vi "Get Modification Flags.vi"(8 "error in (no error)":errorcluster, 10 "Saved Item in":refnum<class "Item.lvclass">, 11 "Item in":refnum<class "Item.lvclass">) -> (0 "error out":errorcluster, 1 "Modification Flags":bool[](array[boolean]), 2 "Saved Item out":refnum<class "Item.lvclass">, 3 "Item out":refnum<class "Item.lvclass">)   [LabVIEW 2020, in "VI Properties Editor.lvlib" / "Item.lvclass"]
doc: "Gets the modification flags of <B>Item in</B> by comparing it to <B>Saved Item in</B>."
uses:
  Item.lvclass
  <vilib>/LabVIEW Icon API/lv_icon/Classes/Icon/Icon.lvclass
  Item.lvclass/Item.ctl
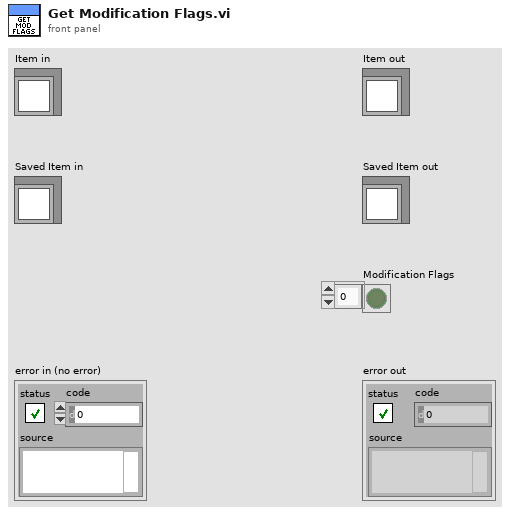
[diagram p1: front panel]
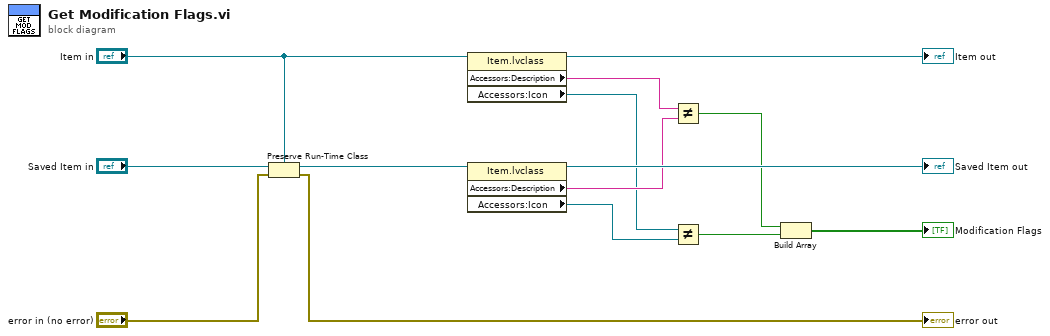
[diagram p0: block diagram]
diagram:
  n1 = Preserve Run-Time Class(object in="Saved Item in", error in="error in (no error)", 2:"Item in") -> (object out=w8:refnum<class "Item.lvclass">, error out=→"error out":errorcluster)
  n2 = property class="Item.lvclass"(reference="Item in") -> (reference out=→"Item out":refnum<class "Item.lvclass">, "Accessors:Description"=w7:string, "Accessors:Icon"=w5:refnum<class "Icon.lvclass">)  [unwired: 1 in, 1 out]
  n3 = property class="Item.lvclass"(reference=w8) -> (reference out=→"Saved Item out":refnum<class "Item.lvclass">, "Accessors:Description"=w6:string, "Accessors:Icon"=w4:refnum<class "Icon.lvclass">)  [unwired: 1 in, 1 out]
  n4 = Not Equal?(x=w7, y=w6) -> (x != y?=w3:bool)
  n5 = Not Equal?(x=w5, y=w4) -> (x != y?=w2:bool)
  n6 = Build Array(w3, w2) -> (→"Modification Flags":bool[])
